vi "具体消息显示.vi"(2 "error in (no error)":errorcluster caption="错误输入（无错误）", 3 "ID":dbl) -> (1 "html_url":string)   [LabVIEW 2012]
uses:
  <vilib>/addons/WireFlow/_WF_ProgressBar.llb/MessageTextType.ctl
  <vilib>/addons/WireFlow/_WF_ProgressBar.llb/ProgressBar_WireFlow.lvclass
panel:
  in  "delay (0 ms)":i32=1000
  out "error out":errorcluster
  out "字符串":string
  in  "WebBrowser":refnum<k7>(container) caption="网页浏览器"
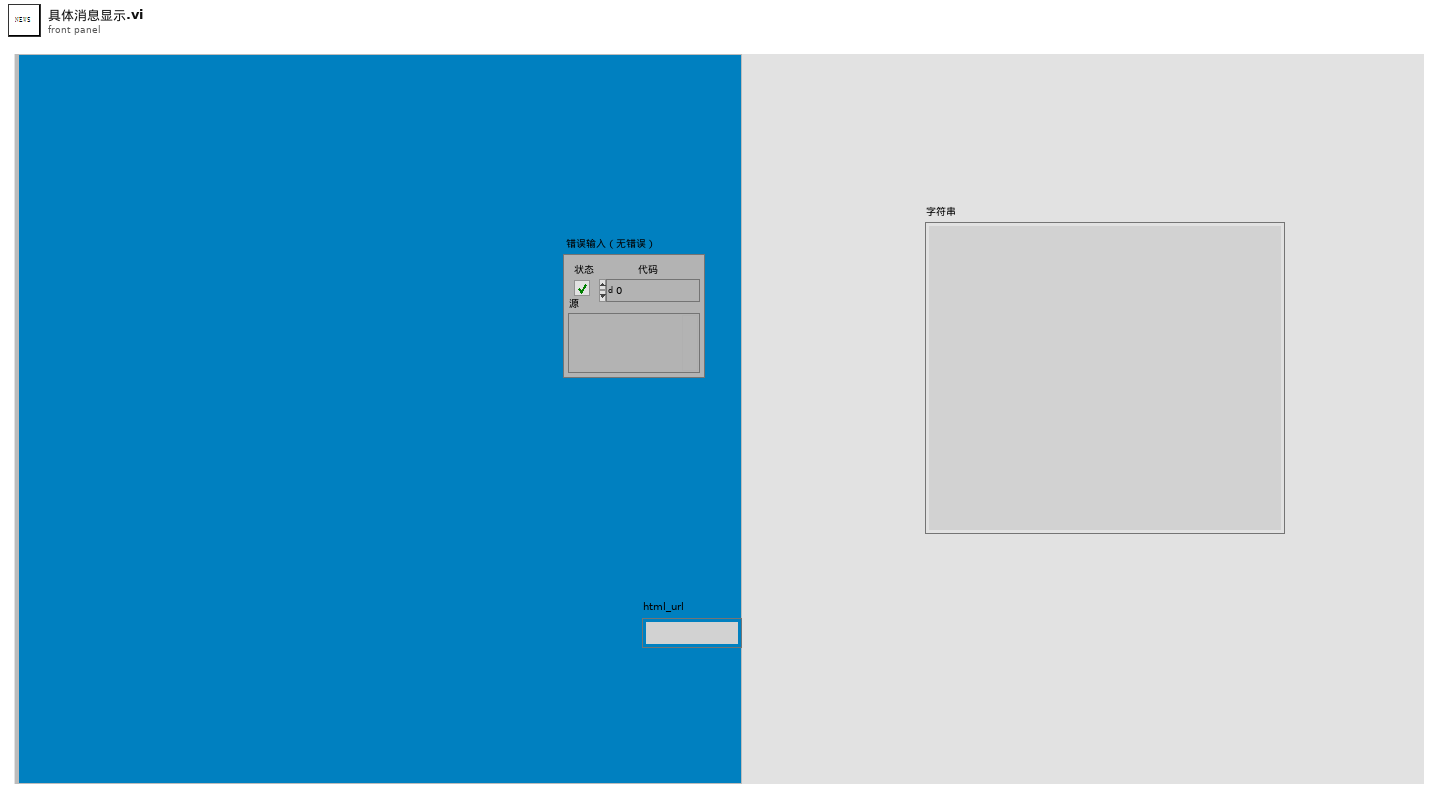
[diagram p1: front panel]
types:
  T1 = typedef "ProgressBar_WireFlow.lvclass/MessageTextType.ctl" = enum16{"Title", "General", "Current item"}
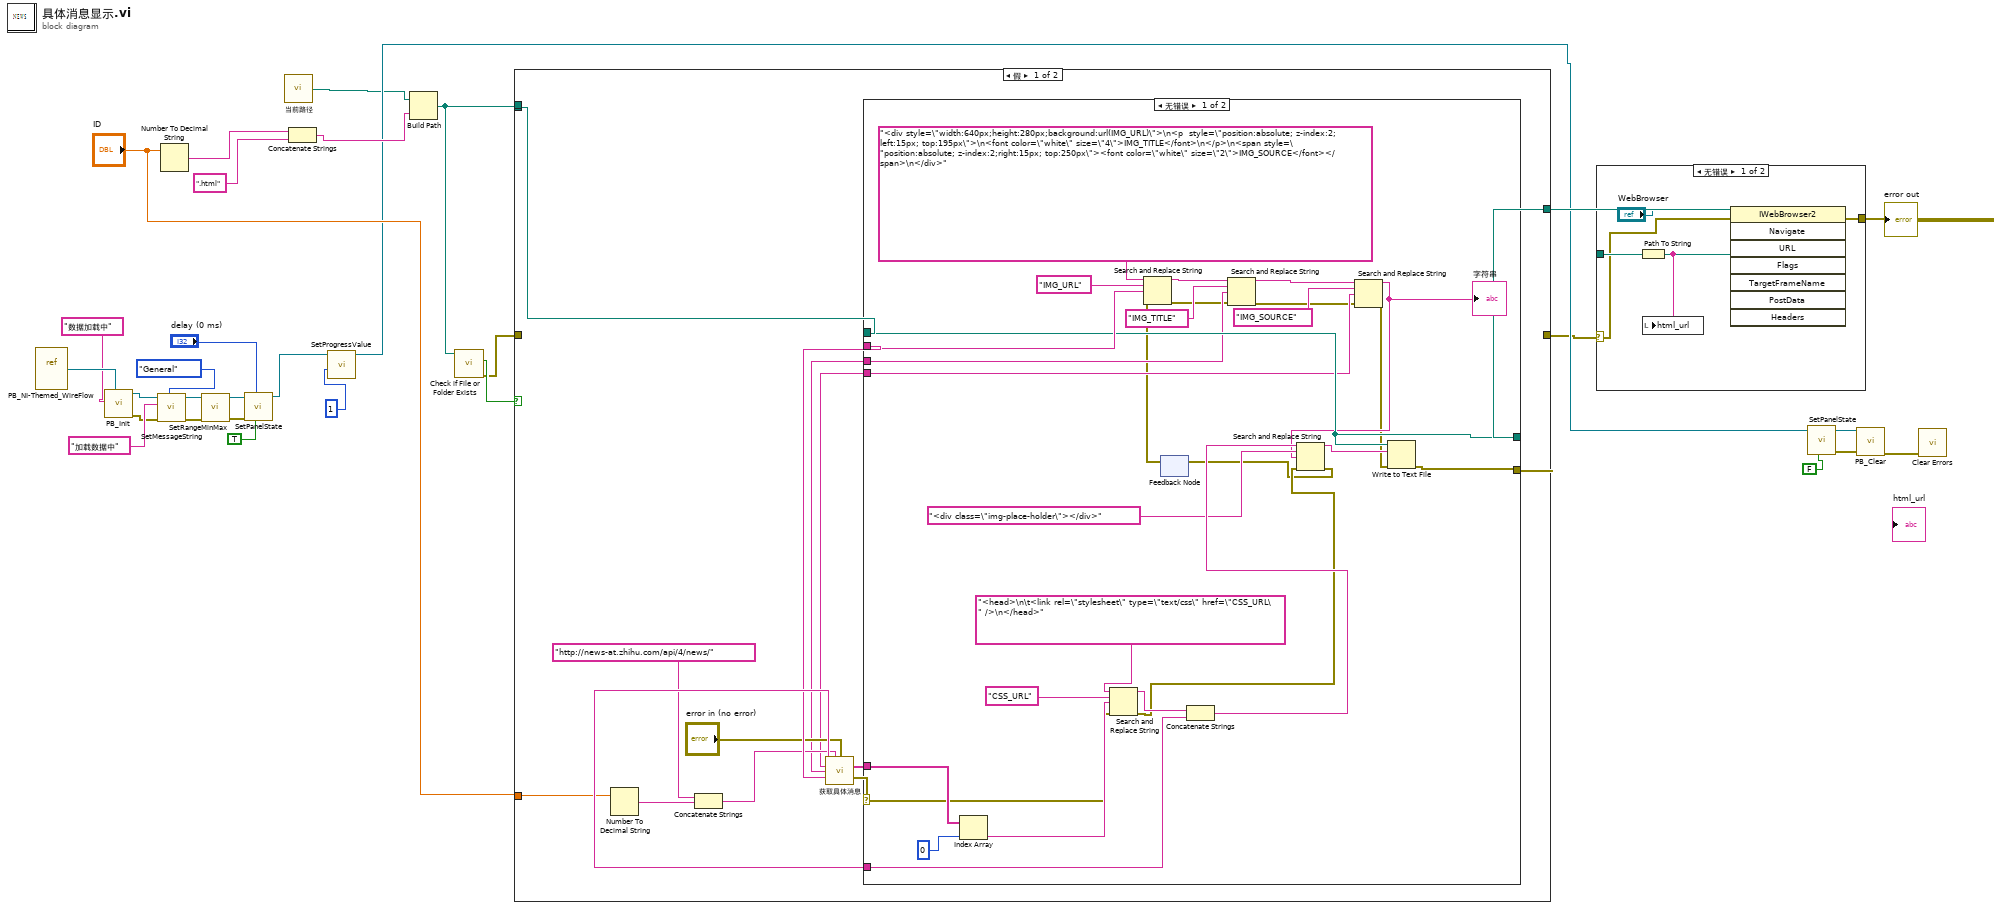
[diagram p0: block diagram]
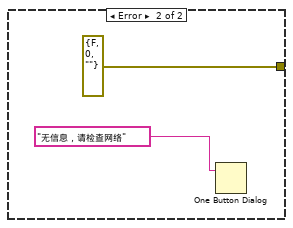
[diagram p2: hidden frame]
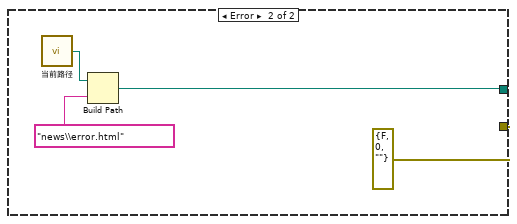
[diagram p3: hidden frame]
diagram:
  n1 = vi-ref "PB_NI-Themed_WireFlow.vi"() -> (w23:refnum<vi>)
  n2 = call <vilib>:"PB_Init.vi"("Progress VI"=w23, "title (\"Progress\")"="数据加载中") -> ("error out"=w16:errorcluster, "WF-ProgressBar out"=w21:refnum<class "ProgressBar_WireFlow.lvclass">)  [unwired: 8 in]
  n3 = call-dynamic "SetMessageString.vi"("message field"=MessageTextType."General", "error in (no error)"=w16, "Message"="加载数据中", "WF-ProgressBar in"=w21) -> ("error out"=w17:errorcluster, "WF-ProgressBar out"=w18:refnum<class "ProgressBar_WireFlow.lvclass">)  [unwired: 6 in]
  n4 = Number To Decimal String(number="ID") -> (decimal integer string=w2:string)  [unwired: 1 in]
  n5 = call-dynamic "SetRangeMinMax.vi"("error in (no error)"=w17, "WF-ProgressBar in"=w18) -> ("error out"=w14:errorcluster, "WF-ProgressBar out"=w15:refnum<class "ProgressBar_WireFlow.lvclass">)  [unwired: 8 in]
  n6 = call-dynamic "SetPanelState.vi"("State (T = Open)"=TRUE, "delay (0 ms)"="delay (0 ms)", "error in (no error)"=w14, "WF-ProgressBar in"=w15) -> ("WF-ProgressBar out"=w11:refnum<class "ProgressBar_WireFlow.lvclass">)  [unwired: 6 in, 1 out]
  n7 = call "当前路径.vi"() -> ("路径"=w5:path)
  n8 = Concatenate Strings(w2, ".html") -> (w30:string)
  n9 = call-dynamic "SetProgressValue.vi"("Value"=1, "WF-ProgressBar in"=w11) -> ("WF-ProgressBar out"=w6:refnum<class "ProgressBar_WireFlow.lvclass">)  [unwired: 7 in, 2 out]
  n10 = Build Path(base path=w5, name or relative path=w30) -> (appended path=w29:path)
  n11 = call <vilib>:"Check if File or Folder Exists.vi"("path"=w29) -> ("error out"=w26:errorcluster, "file or folder exists?"=w28:bool)  [unwired: 8 in, 1 out]
  n12 = case shown="假" w28 {
    tunnel: "ID" -> [w36 _]
    tunnel: w29 -> [w34 w79]
    tunnel: w29 -> [_ _]
    tunnel: [w35 w79] -> w27
    tunnel: [w31 w78] -> w4
    tunnel: w26 -> [_ w78]
    frame False {
      n13 = Number To Decimal String(number=w36) -> (decimal integer string=w41:string)  [unwired: 1 in]
      n14 = Concatenate Strings("http://news-at.zhihu.com/api/4/news/", w41) -> (w39:string)
      n15 = call "获取具体消息.vi"("URL"=w39, "error in (no error)"="error in (no error)") -> ("body"=w43:string, "image_source"=w32:string, "css"=w44:string[], "title"=w33:string, "image"=w42:string, "error out"=w37:errorcluster)  [unwired: 2 in, 6 out]
      n16 = case shown="无错误" w37 {
        selector: w37 -> [w51 _]
        tunnel: w44 -> [w64 _]
        tunnel: w43 -> [w63 _]
        tunnel: w42 -> [w62 _]
        tunnel: w34 -> [w60 _]
        tunnel: [w59 errorcluster {"status"=FALSE, "code"=0, "source"=""} ("错误常量")] -> w31
        tunnel: [w60 w74] -> w35
        tunnel: w33 -> [w56 _]
        tunnel: w32 -> [w53 _]
        frame No Error {
          n17 = Index Array(array=w64, index=0) -> (element=w71:string)
          n18 = Search and Replace String(input string="<head>\n\t<link rel=\"stylesheet\" type=\"text/css\" href=\"CSS_URL\" />\n</head>", search string="CSS_URL", replace string=w71, error in=w51) -> (result string=w69:string, error out=w50:errorcluster)  [unwired: 4 in, 2 out]
          n19 = feedback #1() -> (w45:errorcluster)  [unwired: 1 in]
          n20 = Search and Replace String(input string="<div style=\"width:640px;height:280px;background:url(IMG_URL)\">\n<p  style=\"position:absolute; z-index:2; left:15px; top:195px\">\n<font color=\"white\" size=\"4\">IMG_TITLE</font>\n</p>\n<span style=\"position:absolute; z-index:2;right:15px; top:250px\"><font color=\"white\" size=\"2\">IMG_SOURCE</font></span>\n</div>", search string="IMG_URL", replace string=w62, error in=w45) -> (result string=w58:string, error out=w49:errorcluster)  [unwired: 4 in, 2 out]
          n21 = Concatenate Strings(w69, w63) -> (w66:string)
          n22 = Search and Replace String(input string=w58, search string="IMG_TITLE", replace string=w56, error in=w49) -> (result string=w55:string, error out=w48:errorcluster)  [unwired: 4 in, 2 out]
          n23 = Search and Replace String(input string=w55, search string="IMG_SOURCE", replace string=w53, error in=w48) -> (result string=w52:string, error out=w47:errorcluster)  [unwired: 4 in, 2 out]
          "字符串" <- w52
          n24 = Search and Replace String(input string=w66, search string="<div class=\"img-place-holder\"></div>", replace string=w52, error in=w50) -> (result string=w61:string, error out=w46:errorcluster)  [unwired: 4 in, 2 out]
          n25 = feedback-in #1(w46) -> ()
          n26 = Write to Text File(file (use dialog)=w60, text=w61, error in=w47) -> (error out=w59:errorcluster)  [unwired: 1 in, 2 out]
        }
        frame Error {
          n27 = call "当前路径.vi"() -> ("路径"=w75:path)
          n28 = Build Path(base path=w75, name or relative path="news\\error.html") -> (appended path=w74:path)
        }
      }
    }
    frame True {
    }
  }
  n29 = case shown="无错误" w4 {
    selector: w4 -> [w80 _]
    tunnel: w27 -> [w84 _]
    tunnel: [w83 errorcluster {"status"=FALSE, "code"=0, "source"=""} ("错误常量")] -> w24
    frame No Error {
      n30 = Path To String(path=w84) -> (string=w82:string)
      n31 = local write "html_url"(w82) -> ()
      n32 = invoke class="IWebBrowser2" method="Navigate"(reference="WebBrowser", error in=w80, "URL"=w82) -> (error out=w83:errorcluster)  [unwired: 5 in, 7 out]
    }
    frame Error {
      n33 = One Button Dialog(message="无信息，请检查网络") -> ()  [unwired: 1 in, 1 out]
    }
  }
  "error out" <- w24
  n34 = call-dynamic "SetPanelState.vi"("State (T = Open)"=FALSE, "WF-ProgressBar in"=w6) -> ("error out"=w8:errorcluster, "WF-ProgressBar out"=w9:refnum<class "ProgressBar_WireFlow.lvclass">)  [unwired: 8 in]
  n35 = call-dynamic "PB_Clear.vi"("error in (no error)"=w8, "WF-ProgressBar in"=w9) -> ("error out"=w3:errorcluster)  [unwired: 8 in, 1 out]
  n36 = call <vilib>:"Clear Errors.vi"("error in (no error)"=w3) -> ()  [unwired: 6 in, 1 out]
